vi "Write Test VIs.vi"(8 "error in (no error)":errorcluster, 10 "Test VIs":path[](array[path]), 11 "Test Runner in":refnum<class "Test Runner.lvclass">) -> (0 "error out":errorcluster, 3 "Test Runner out":refnum<class "Test Runner.lvclass">)   [LabVIEW 2020, in "Caraya.lvlib" / "Test Runner.lvclass"]
uses:
  Test Runner.lvclass
  Test Runner.lvclass/Test Runner.ctl
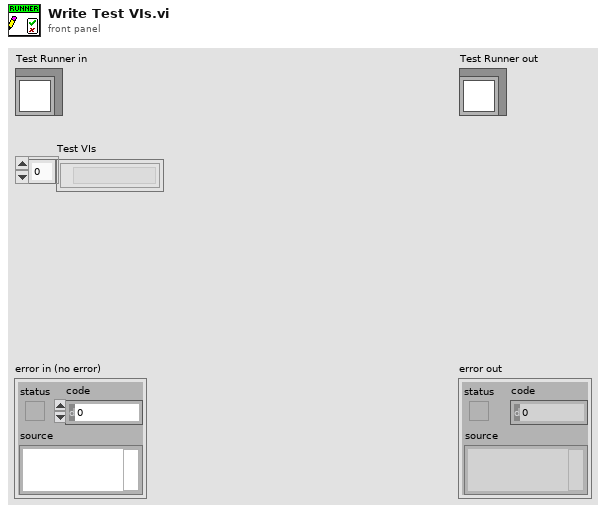
[diagram p1: front panel]
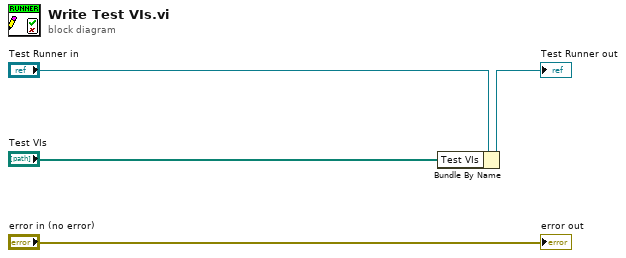
[diagram p0: block diagram]
diagram:
  n1 = Bundle By Name(cluster="Test Runner in", "Test VIs"="Test VIs") -> (→"Test Runner out":refnum<class "Test Runner.lvclass">)
  "error out" <- "error in (no error)"
